vi "Update Layout.vi"(6 "Sync Response":refnum<notifier>, 8 "error in (no error)":errorcluster, 10 "Synced":bool, 11 "2DArrayManager in":refnum<class "2DArrayManager.lvclass">) -> (0 "error out":errorcluster, 3 "2DArrayManager out":refnum<class "2DArrayManager.lvclass">)   [LabVIEW 2020, in "OOPanel.lvlib" / "2DArrayManager.lvclass"]
uses:
  2DArrayManager.lvclass
  2DArrayManager.lvclass/2DArrayManager.ctl
  2DPanelBlank/2DPanelBlank.lvclass/2DPanelBlank.ctl
  2DPanelBlank/Get Info.vi
  2DPanelBlank/Clear Position.vi
  2DPanelBlank/2DPanelBlank.lvclass
  C:/dev/lv20CE/relink/lv-oopanel/OOPanel/Panel/Panel.lvclass
  Close All Blanks.vi
  Manager/Create Panel by Type.vi
  Manager/Get Panel from SubPanel.vi
  Manager/Remove Panel from SubPanel.vi
  ArrayPanel/ArrayPanel.lvclass
panel:
  out "Name":string
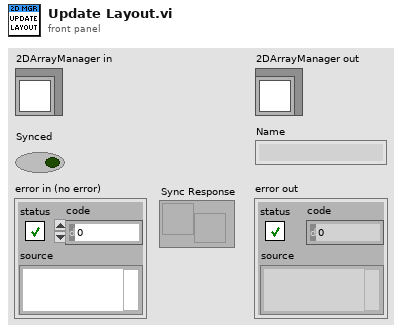
[diagram p1: front panel]
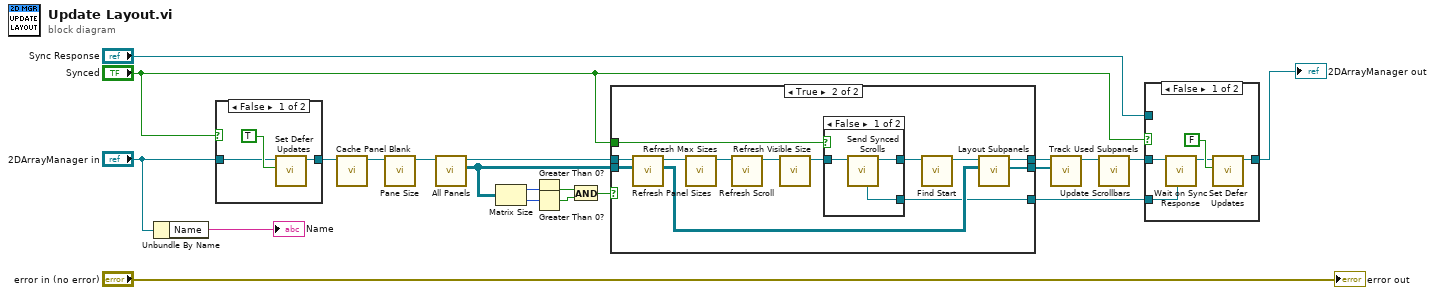
[diagram p0: block diagram]
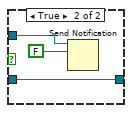
[diagram p5: hidden frame]
diagram:
  n1 = Unbundle By Name("2DArrayManager in") -> ("Name"=→"Name":string)
  n2 = case shown="False" "Synced" {
    tunnel: "2DArrayManager in" -> [w23 w25]
    tunnel: [w22 w25] -> w20
    frame False {
      n3 = call "Set Defer Updates.vi"("Defer Updates"=TRUE, "2DArrayManager in"=w23) -> ("2DArrayManager out"=w22:refnum<class "2DArrayManager.lvclass">)  [unwired: 8 in, 1 out]
    }
    frame True {
    }
  }
  n4 = call "Cache Panel Blank.vi"("2DArrayManager in"=w20) -> ("2DArrayManager out"=w4:refnum<class "2DArrayManager.lvclass">)  [unwired: 9 in, 1 out]
  n5 = call "Pane Size.vi"("2DArrayManager in"=w4) -> ("2DArrayManager out"=w12:refnum<class "2DArrayManager.lvclass">)  [unwired: 9 in, 1 out]
  n6 = call "All Panels.vi"("2DArrayManager in"=w12) -> ("Panels"=w13:refnum<class "ArrayPanel.lvclass">[][], "2DArrayManager out"=w14:refnum<class "2DArrayManager.lvclass">)  [unwired: 8 in, 1 out]
  n7 = Matrix Size(0:w13) -> (1:w19:i32, 2:w18:i32)
  n8 = Greater Than 0?(x=w19) -> (x > 0?=w17:bool)
  n9 = Greater Than 0?(x=w18) -> (x > 0?=w16:bool)
  n10 = And(x=w17, y=w16) -> (x .and. y?=w15:bool)
  n11 = case shown="True" w15 {
    tunnel: w14 -> [w26 w39]
    tunnel: w13 -> [_ w38]
    tunnel: [w26 w33] -> w7
    tunnel: "Synced" -> [_ w32]
    tunnel: [_ w29] -> w9
    tunnel: [_ w28] -> w5
    frame False {
    }
    frame True {
      n12 = call "Refresh Panel Sizes.vi"("Panels in"=w38, "2DArrayManager in"=w39) -> ("Panels"=w34:refnum<class "ArrayPanel.lvclass">[][], "2DArrayManager out"=w37:refnum<class "2DArrayManager.lvclass">)  [unwired: 7 in, 1 out]
      n13 = call "Refresh Max Sizes.vi"("2DArrayManager in"=w37) -> ("2DArrayManager out"=w36:refnum<class "2DArrayManager.lvclass">)  [unwired: 9 in, 1 out]
      n14 = call "Refresh Scroll.vi"("2DArrayManager in"=w36) -> ("2DArrayManager out"=w31:refnum<class "2DArrayManager.lvclass">)  [unwired: 9 in, 1 out]
      n15 = call "Refresh Visible Size.vi"("2DArrayManager in"=w31) -> ("2DArrayManager out"=w27:refnum<class "2DArrayManager.lvclass">)  [unwired: 9 in, 1 out]
      n16 = case shown="False" w32 {
        tunnel: w27 -> [w42 w43]
        tunnel: [w41 w43] -> w30
        tunnel: [w40 _] -> w29
        frame False {
          n17 = call "Send Synced Scrolls.vi"("2DArrayManager in"=w42) -> ("2DArrayManager out"=w41:refnum<class "2DArrayManager.lvclass">, "Sync Response"=w40:refnum<notifier>)  [unwired: 8 in, 1 out]
        }
        frame True {
        }
      }
      n18 = call "Find Start.vi"("2DArrayManager in"=w30) -> ("2DArrayManager out"=w35:refnum<class "2DArrayManager.lvclass">)  [unwired: 9 in, 1 out]
      n19 = call "Layout Subpanels.vi"("Panels in"=w34, "2DArrayManager in"=w35) -> ("Used SubPanels"=w28:refnum<vi>[], "2DArrayManager out"=w33:refnum<class "2DArrayManager.lvclass">)  [unwired: 6 in, 2 out]
    }
  }
  n20 = call "Track Used Subpanels.vi"("Used SubPanels"=w5, "2DArrayManager in"=w7) -> ("2DArrayManager out"=w6:refnum<class "2DArrayManager.lvclass">)  [unwired: 8 in, 1 out]
  n21 = call "Update Scrollbars.vi"("2DArrayManager in"=w6) -> ("2DArrayManager out"=w11:refnum<class "2DArrayManager.lvclass">)  [unwired: 9 in, 1 out]
  n22 = case shown="False" "Synced" {
    tunnel: [w48 w51] -> w2
    tunnel: w11 -> [w46 w51]
    tunnel: w9 -> [w44 _]
    tunnel: "Sync Response" -> [_ w49]
    frame False {
      n23 = call "Wait on Sync Response.vi"("Sync Response"=w44, "2DArrayManager in"=w46) -> ("2DArrayManager out"=w45:refnum<class "2DArrayManager.lvclass">)  [unwired: 8 in, 1 out]
      n24 = call "Set Defer Updates.vi"("Defer Updates"=FALSE, "2DArrayManager in"=w45) -> ("2DArrayManager out"=w48:refnum<class "2DArrayManager.lvclass">)  [unwired: 8 in, 1 out]
    }
    frame True {
      n25 = Send Notification(notification=FALSE, notifier=w49) -> ()  [unwired: 1 in, 2 out]
    }
  }
  "2DArrayManager out" <- w2
  "error out" <- "error in (no error)"
